vi "CreateCommandWrapperMac.vi"() -> ()   [LabVIEW 2026]
doc: "Creates a reentrant command wrapper. Wires all subVI inputs/outputs to named controls/indicators. No connector assignments. Never executes the command."
uses:
  <vilib>/Utility/miscctls.llb/LVPointTypeDef.ctl
panel:
  out "error out":errorcluster
  out "terminal errors":errorcluster[](array[cluster])
  in  "project path":string
  in  "terminal numbers":dbl[](array[numeric])
  in  "wrapper path":string
  in  "command path":string
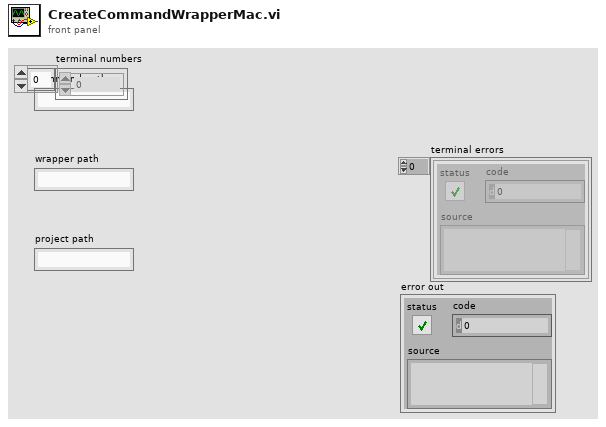
[diagram p1: front panel]
types:
  T1 = typedef "LVPointTypeDef.ctl" = cluster{"Horizontal":i16, "Vertical":i16}
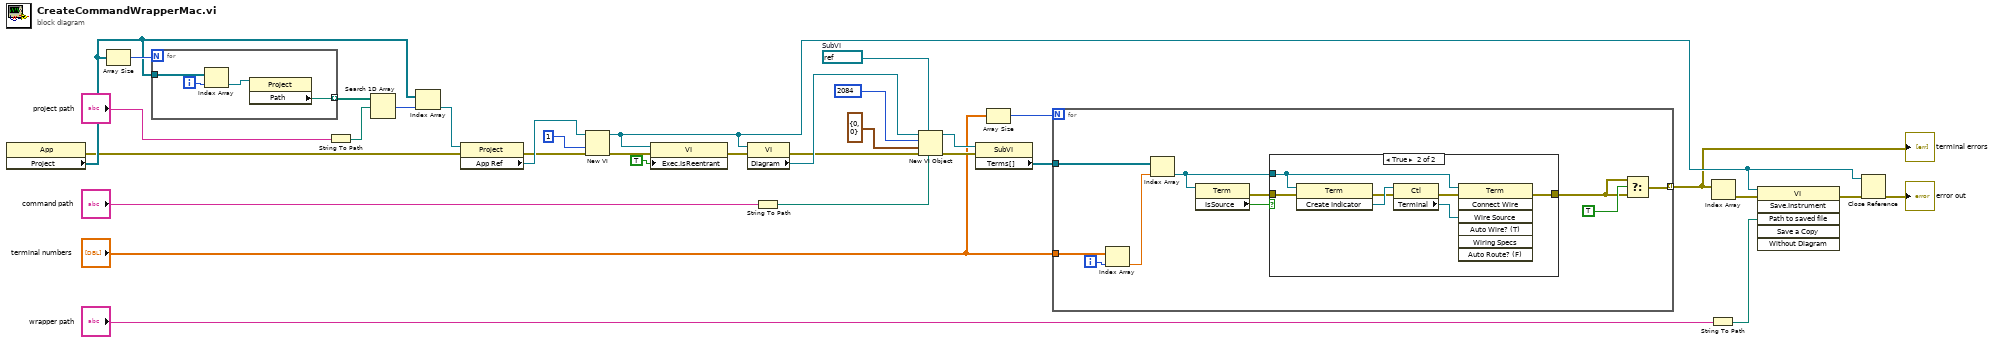
[diagram p0: block diagram]
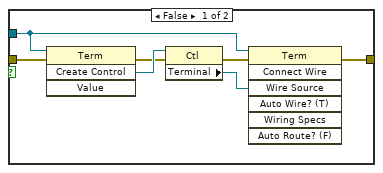
[diagram p2: hidden frame]
diagram:
  w16 = refnum<vi> refnum  # SubVI
  n1 = property class="App"() -> (error out=w24:errorcluster, "Project"=w30:refnum<vi>[])  [unwired: 2 in, 1 out]
  n2 = Array Size(array=w30) -> (size(s)=w31:i32)
  n3 = for {
    N: w31 -> [_]
    tunnel: w30 -> [w37]
    tunnel: [w34] -> w27 mode=indexing
    i -> [w36]
    n4 = Index Array(array=w37, index=w36) -> (element=w35:refnum<vi>)
    n5 = property class="Project"(reference=w35) -> ("Path"=w34:path)  [unwired: 1 in, 2 out]
  }
  n6 = String To Path(string="project path") -> (path=w28:path)
  n7 = Search 1D Array(1D array=w27, element=w28) -> (index of element=w26:i32)  [unwired: 1 in]
  n8 = Index Array(array=w30, index=w26) -> (element=w25:refnum<vi>)
  n9 = property class="Project"(reference=w25, error in=w24) -> (error out=w22:errorcluster, "App Ref"=w23:refnum<vi>)  [unwired: 1 out]
  n10 = New VI(8:w22, 9:1, 11:w23) -> (0:w19:errorcluster, 3:w20:refnum<vi>)  [unwired: 4 in]
  n11 = property class="VI"(reference=w20, error in=w19, "Exec.IsReentrant"=TRUE) -> (error out=w17:errorcluster)  [unwired: 1 out]
  n12 = property class="VI"(reference=w20, error in=w17) -> (error out=w13:errorcluster, "Diagram"=w14:refnum<vi>)  [unwired: 1 out]
  n13 = String To Path(string="command path") -> (path=w12:path)
  n14 = New VI Object(vi object class=w16, owner refnum=w14, style=u32 2084, position/next to=T1 {"Horizontal"=0, "Vertical"=0} ("location"), 6:w12, 8:w13) -> (object refnum=w10:refnum<vi>, 0:w9:errorcluster)  [unwired: 2 in]
  n15 = property class="SubVI"(reference=w10, error in=w9) -> ("Terms[]"=w6:refnum<vi>[])  [unwired: 2 out]
  n16 = Array Size(array="terminal numbers") -> (size(s)=w8:i32)
  n17 = for {
    N: w8 -> [_]
    tunnel: "terminal numbers" -> [w47]
    tunnel: w6 -> [w45]
    tunnel: [w38] -> w5 mode=indexing
    i -> [w46]
    n18 = Index Array(array=w47, index=w46) -> (element=w44:dbl)
    n19 = Index Array(array=w45, index=w44) -> (element=w42:refnum<vi>)
    n20 = property class="Term"(reference=w42) -> (error out=w41:errorcluster, "IsSource"=w43:bool)  [unwired: 1 in, 1 out]
    n21 = case shown="True" w43 {
      tunnel: w42 -> [w54 w61]
      tunnel: w41 -> [w53 w60]
      tunnel: [w48 w55] -> w39
      frame False {
        n22 = invoke class="Term" method="Create Control"(reference=w54, error in=w53) -> (error out=w51:errorcluster, "Create Control"=w52:refnum<vi>)  [unwired: 2 in, 2 out]
        n23 = property class="Ctl"(reference=w52, error in=w51) -> (error out=w50:errorcluster, "Terminal"=w49:refnum<vi>)  [unwired: 1 out]
        n24 = invoke class="Term" method="Connect Wire"(reference=w54, error in=w50, "Wire Source"=w49) -> (error out=w48:errorcluster)  [unwired: 4 in, 6 out]
      }
      frame True {
        n25 = invoke class="Term" method="Create Indicator"(reference=w61, error in=w60) -> (error out=w58:errorcluster, "Create Indicator"=w59:refnum<vi>)  [unwired: 1 in, 1 out]
        n26 = property class="Ctl"(reference=w59, error in=w58) -> (error out=w57:errorcluster, "Terminal"=w56:refnum<vi>)  [unwired: 1 out]
        n27 = invoke class="Term" method="Connect Wire"(reference=w61, error in=w57, "Wire Source"=w56) -> (error out=w55:errorcluster)  [unwired: 4 in, 6 out]
      }
    }
    n28 = Select(t=w39, s=TRUE, f=w39) -> (s? t:f=w38:errorcluster)
  }
  "terminal errors" <- w5
  n29 = String To Path(string="wrapper path") -> (path=w3:path)
  n30 = Index Array(array=w5) -> (element=w4:errorcluster)  [unwired: 1 in]
  n31 = invoke class="VI" method="Save.Instrument"(reference=w20, error in=w4, "Path to saved file"=w3) -> (error out=w2:errorcluster)  [unwired: 3 in, 5 out]
  n32 = Close Reference(reference=w20, error in (no error)=w2) -> (error out=→"error out":errorcluster)
